vi "Connect Call Box.vi"(8 "error in (no error)":errorcluster caption="에러 입력(에러 없음)", 10 "VISA Address":refnum<visa-resource-name>, 11 "Instrument Manager 입력":refnum<class "Instrument Manager.lvclass">) -> (0 "error out":errorcluster caption="에러 출력", 3 "Instrument Manager 출력":refnum<class "Instrument Manager.lvclass">)   [LabVIEW 2023, in "Instrument Manager.lvclass"]
uses:
  Instrument Manager.lvclass
  Module/ANRITSU Call Box/Implement Class/Anritsu Call Box_Implement/Anritsu Call Box_Implement.lvclass
  Module/ANRITSU Call Box/Type Definition/Call Device - Protocol Type Selector.ctl
  Instrument Manager.lvclass/Instrument Manager.ctl
  Module/ANRITSU Call Box/ANRITSU Call Box.lvlib
  C:/Users/HCT-3320/Documents/Instrument Manger/Module/ANRITSU Call Box/Implement Class/Anritsu Call Box_Implement/Anritsu Call Box_Implement.lvclass
  C:/Users/HCT-3320/Documents/Instrument Manger/Module/ANRITSU Call Box/Interface Class/Anritsu Call Box.lvclass
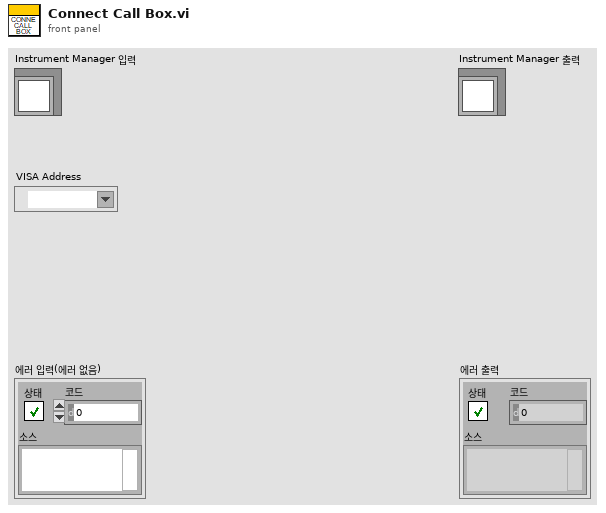
[diagram p1: front panel]
types:
  T1 = typedef "ANRITSU Call Box.lvlib/Call Device - Protocol Type Selector.ctl" = enum16{"8000A - NR", "8000A - LTE", "882xC - LTE"}
  T2 = cluster{"Anritsu Call Box":refnum<class "Anritsu Call Box.lvclass">, "Spectrum Analyzer":refnum<class "Interface_Spectrum.lvclass">, "RF Switch Box":refnum<class "RF Filter Box.lvclass">, "Turn Table":refnum<class "Interface - Turn Table.lvclass">, "Mast":refnum<class "Interface - Mast.lvclass">, "3D Controller":refnum<class "Interface_3D Controller.lvclass">}
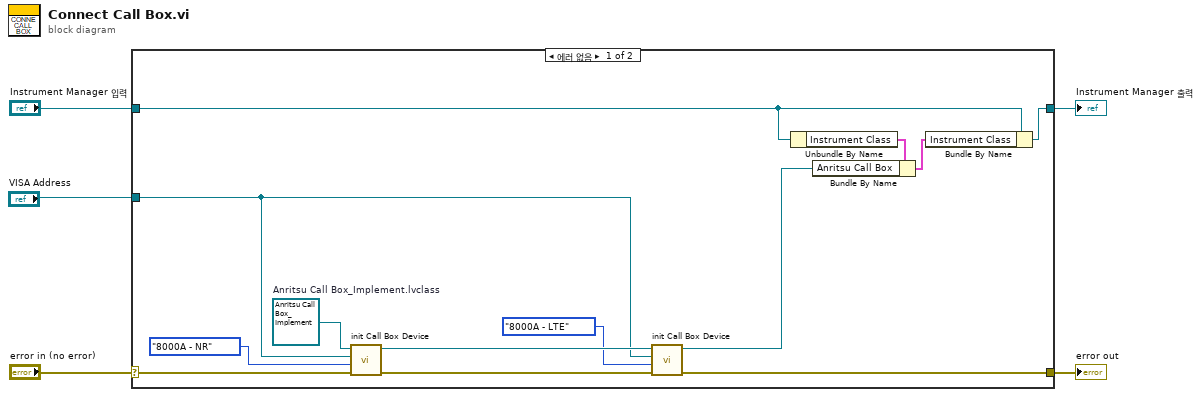
[diagram p0: block diagram]
diagram:
  n1 = case shown="에러 없음" "error in (no error)" {
    selector: "error in (no error)" -> [w14 w20]
    tunnel: [w7 w20] -> w4
    tunnel: [w17 w19] -> w2
    tunnel: "Instrument Manager 입력" -> [w18 w19]
    tunnel: "VISA Address" -> [w6 _]
    frame No Error {
      w12 = refnum<class "Anritsu Call Box_Implement.lvclass"> refnum  # Anritsu Call Box_Implement.lvclass
      n2 = call-dynamic "init Call Box Device.vi"("error in (no error)"=w14, "Device - Protocol"=Call_Device_-_Protocol_Type_Selector."8000A - NR", "VISA Address"=w6, "Anritsu Call Box_Implement in"=w12) -> ("error out"=w11:errorcluster, "Anritsu Call Box_Implement out"=w10:refnum<class "Anritsu Call Box_Implement.lvclass">)  [unwired: 5 in, 1 out]
      n3 = call-dynamic "init Call Box Device.vi"("error in (no error)"=w11, "Device - Protocol"=Call_Device_-_Protocol_Type_Selector."8000A - LTE", "VISA Address"=w6, "Anritsu Call Box_Implement in"=w10) -> ("error out"=w7:errorcluster, "Anritsu Call Box_Implement out"=w8:refnum<class "Anritsu Call Box_Implement.lvclass">)  [unwired: 5 in, 1 out]
      n4 = Unbundle By Name(w18) -> ("Instrument Class"=w16:T2)
      n5 = Bundle By Name(cluster=w16, "Anritsu Call Box"=w8) -> (w15:T2)
      n6 = Bundle By Name(cluster=w18, "Instrument Class"=w15) -> (w17:refnum<class "Instrument Manager.lvclass">)
    }
    frame Error {
    }
  }
  "error out" <- w4
  "Instrument Manager 출력" <- w2
